vi "Measure_Voltage.vi"(6 "Resolution in Digits":T1(ring), 8 "error in (no error)":errorcluster, 9 "Range":dbl=1.2, 10 "Level":dbl=1.2, 11 "NI-DCPower in":refnum<class "niDCPower.lvclass">) -> (0 "error out":errorcluster, 1 "Out of Range":bool, 2 "DC_Voltage":dbl, 3 "NI-DCPower out":refnum<class "niDCPower.lvclass">)   [LabVIEW 2021, in "niDCPower.lvclass"]
uses:
  niDCPower.lvclass
  <instrlib>/niDCPower/nidcpower.llb/niDCPower Wait For Event - Event.ctl
  <instrlib>/niDCPower/nidcpower.llb/niDCPower Measurement Type.ctl
  niDCPower.lvclass/niDCPower.ctl
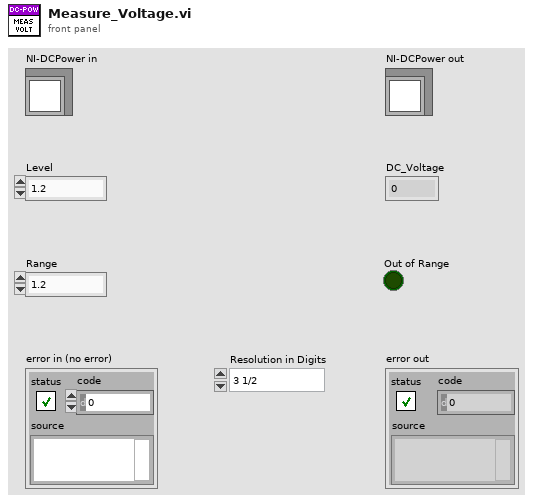
[diagram p1: front panel]
types:
  T1 = enum32{"3 1/2", "4 1/2", "5 1/2", "6 1/2", "7 1/2"}
  T2 = enum32{"DC Volts", "AC Volts", "DC Current", "AC Current", "2-wire Resistance", "4-wire Resistance", "Diode", "Frequency", "Period", "AC Volts DC Coupled", "Capacitance", "Inductance", "Temperature"}
  T3 = typedef "niDCPower Measurement Type.ctl" = i32
  T4 = typedef "niDCPower Wait For Event - Event.ctl" = i32
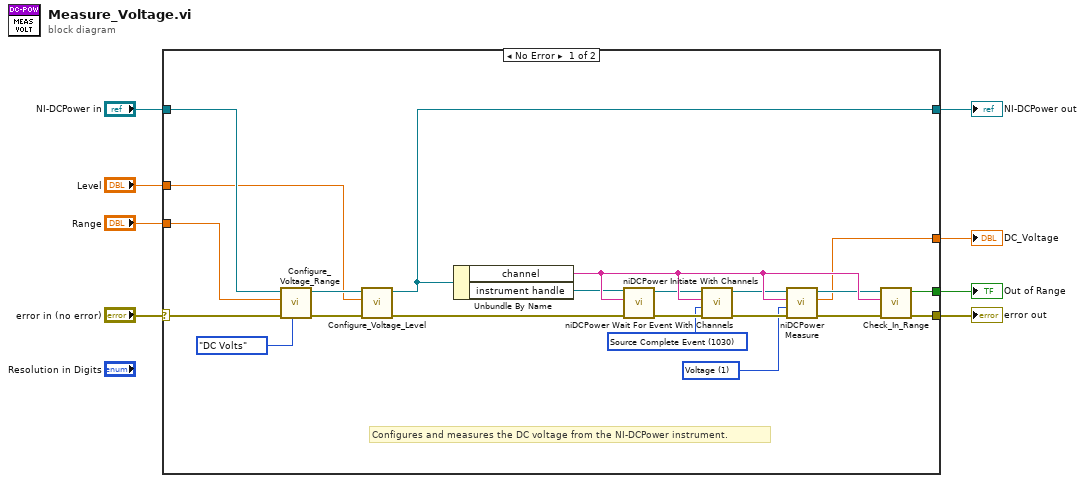
[diagram p0: block diagram]
diagram:
  n1 = case shown="No Error" "error in (no error)" {
    selector: "error in (no error)" -> [w30 w31]
    tunnel: "NI-DCPower in" -> [w12 w32]
    tunnel: [w29 w31] -> w6
    tunnel: [w27 w32] -> w5
    tunnel: "Range" -> [w13 _]
    tunnel: "Level" -> [w11 _]
    tunnel: [w10 _] -> w2
    tunnel: [w9 _] -> w1
    frame No Error {
      w18 = T3 1 items=["Current", "Voltage"] ("measurement type")
      w22 = T4 1030 items=["Source Complete Event"=1030, "Measure Complete Event"=1031, "Sequence Iteration Complete Event"=1032, "Sequence Engine Done Event"=1033, "Pulse Complete Event"=1051, "Ready For Pulse Trigger Event"=1052] ("event")
      # "Configures and measures the DC voltage from the NI-DCPower instrument."
      n2 = call "Configure_Voltage_Range.vi"("Measurement Type"=T2."DC Volts", "error in (no error)"=w30, "Range"=w13, "NI-DCPower in"=w12) -> ("error out"=w16:errorcluster, "NI-DCpower out"=w15:refnum<class "niDCPower.lvclass">)  [unwired: 6 in]
      n3 = call "Configure_Voltage_Level.vi"("error in (no error)"=w16, "Level"=w11, "NI-DCPower in"=w15) -> ("error out"=w28:errorcluster, "NI-DCPower out"=w27:refnum<class "niDCPower.lvclass">)  [unwired: 7 in]
      n4 = Unbundle By Name(w27) -> ("channel"=w26:string, "instrument handle"=w25:refnum<k15>)
      n5 = call <instrlib>:"niDCPower Initiate With Channels.vi"("error in (no error)"=w28, "channel name"=w26, "instrument handle"=w25) -> ("error out"=w23:errorcluster, "instrument handle out"=w24:refnum<k15>)  [unwired: 7 in]
      n6 = call <instrlib>:"niDCPower Wait For Event With Channels.vi"("error in (no error)"=w23, "event"=w22, "channel name"=w26, "instrument handle"=w24) -> ("error out"=w21:errorcluster, "instrument handle out"=w20:refnum<k15>)  [unwired: 6 in]
      n7 = call <instrlib>:"niDCPower Measure.vi"("error in (no error)"=w21, "measurement type"=w18, "channel name"=w26, "instrument handle"=w20) -> ("error out"=w19:errorcluster, "measurement"=w9:dbl, "instrument handle out"=w17:refnum<k15>)  [unwired: 5 in]
      n8 = call "Check_In_Range.vi"("error in (no error)"=w19, "channel name"=w26, "instrument handle"=w17) -> ("error out"=w29:errorcluster, "not in compliance?"=w10:bool)  [unwired: 7 in]
    }
    frame Error {
    }
  }
  "error out" <- w6
  "NI-DCPower out" <- w5
  "DC_Voltage" <- w1
  "Out of Range" <- w2
